vi "Show Value.vi"(8 "error in (no error)":errorcluster caption="错误输入（无错误）", 10 "Coords":T1, 11 "Data Viewer 输入":refnum<class "Data Viewer.lvclass">) -> (0 "error out":errorcluster caption="错误输出", 2 "XY":cluster{"X":dbl, "Y":dbl}, 3 "Data Viewer 输出":refnum<class "Data Viewer.lvclass">)   [LabVIEW 2020, in "Data Viewer.lvlib" / "Data Viewer.lvclass"]
uses:
  Data Viewer.lvclass
  <vilib>/Utility/miscctls.llb/LVPoint32TypeDef.ctl
  Data Viewer.lvclass/Data Viewer.ctl
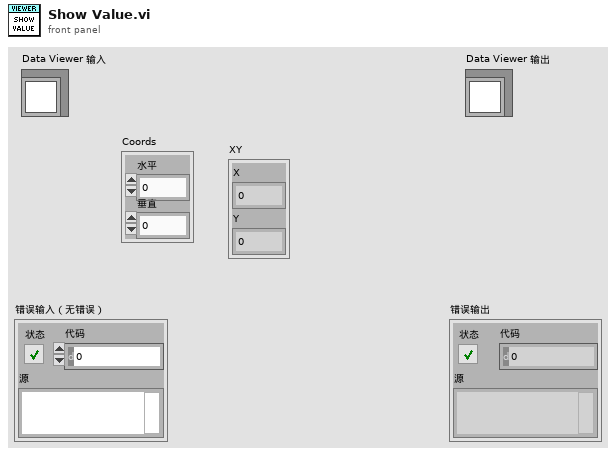
[diagram p1: front panel]
types:
  T1 = typedef "LVPoint32TypeDef.ctl" = cluster{"Horizontal":i32, "Vertical":i32}
  T2 = cluster{"Curve":i32, "Point":cluster{"X":dbl, "Y":dbl}}
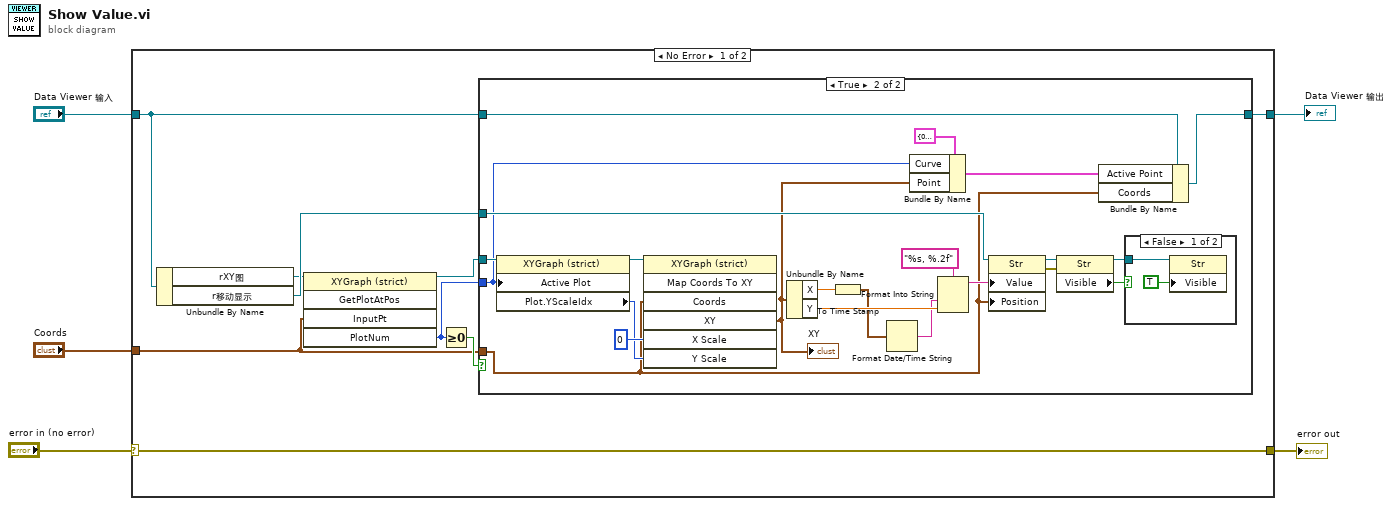
[diagram p0: block diagram]
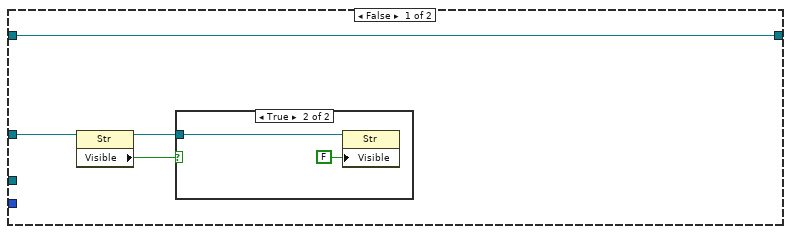
[diagram p2: hidden frame]
diagram:
  n1 = case shown="No Error" "error in (no error)" {
    selector: "error in (no error)" -> [w6 w45]
    tunnel: "Coords" -> [w11 _]
    tunnel: "Data Viewer 输入" -> [w7 w46]
    tunnel: [w6 w45] -> w2
    tunnel: [w8 w46] -> w1
    frame No Error {
      n2 = Unbundle By Name(w7) -> ("rXY图"=w9:refnum<vi>, "r移动显示"=w10:refnum<vi>)
      n3 = invoke class="XYGraph (strict)" method="GetPlotAtPos"(reference=w9, "InputPt"=w11) -> (reference out=w12:refnum<vi>, "PlotNum"=w14:i32)  [unwired: 3 in, 3 out]
      n4 = Greater Or Equal To 0?(x=w14) -> (x >= 0?=w13:bool)
      n5 = case shown="True" w13 {
        tunnel: w12 -> [_ w41]
        tunnel: w14 -> [_ w27]
        tunnel: w11 -> [_ w24]
        tunnel: w10 -> [w18 w35]
        tunnel: [w15 w29] -> w8
        tunnel: w7 -> [w15 w30]
        frame False {
          n6 = property class="Str"(reference=w18) -> (reference out=w17:refnum<vi>, "Visible"=w16:bool)  [unwired: 1 in, 1 out]
          n7 = case shown="True" w16 {
            tunnel: w17 -> [_ w20]
            frame False {
            }
            frame True {
              n8 = property class="Str"(reference=w20, "Visible"=FALSE ("可见")) -> ()  [unwired: 1 in, 2 out]
            }
          }
        }
        frame True {
          n9 = property class="XYGraph (strict)"(reference=w41, "Active Plot"=w27) -> (reference out=w39:refnum<vi>, "Plot.YScaleIdx"=w40:u32)  [unwired: 1 in, 1 out]
          n10 = invoke class="XYGraph (strict)" method="Map Coords To XY"(reference=w39, "Coords"=w24, "X Scale"=0 ("X标尺"), "Y Scale"=w40) -> ("XY"=w26:cluster{"X":dbl, "Y":dbl})  [unwired: 3 in, 6 out]
          "XY" <- w26
          n11 = Unbundle By Name(w26) -> ("X"=w23:dbl, "Y"=w38:dbl)
          n12 = To Time Stamp(1:w23) -> (0:w22:timestamp)
          n13 = Format Date/Time String(seconds (now)=w22) -> (date/time string=w21:string)  [unwired: 2 in]
          n14 = Bundle By Name(cluster=T2 {"Curve"=0, "Point"={"X"=0.0, "Y"=0.0}} ("Active Point"), "Curve"=w27, "Point"=w26) -> (w25:T2)
          n15 = Format Into String(format string="%s, %.2f" ("格式字符串"), w21, w38) -> (resulting string=w36:string)  [unwired: 2 in, 1 out]
          n16 = property class="Str"(reference=w35, "Value"=w36, "Position"=w24) -> (reference out=w34:refnum<vi>, error out=w33:errorcluster)  [unwired: 1 in]
          n17 = property class="Str"(reference=w34, error in=w33) -> (reference out=w31:refnum<vi>, "Visible"=w32:bool)  [unwired: 1 out]
          n18 = Bundle By Name(cluster=w30, "Active Point"=w25, "Coords"=w24) -> (w29:refnum<class "Data Viewer.lvclass">)
          n19 = case shown="False" w32 {
            tunnel: w31 -> [w44 _]
            frame False {
              n20 = property class="Str"(reference=w44, "Visible"=TRUE ("可见")) -> ()  [unwired: 1 in, 2 out]
            }
            frame True {
            }
          }
        }
      }
    }
    frame Error {
    }
  }
  "Data Viewer 输出" <- w1
  "error out" <- w2
